vi "Test Array to Map.vi"() -> ()   [LabVIEW 2020]
uses:
  9a7eb577-90c4-4537-9fff-6973843e9f2b.vi
  9a7eb577-90c4-4537-9fff-6973843e9f2b.vi/b0178052-0c48-4c9a-874f-40b592e34ac5.vi
  <vilib>/addons/_JKI Toolkits/Caraya/classes/Assert/Assert Equal Value and Type_Variant.vi
  <vilib>/addons/_JKI Toolkits/Caraya/classes/Test/Test.lvclass
  <vilib>/addons/_JKI Toolkits/Caraya/classes/Assert/Assert.lvclass
panel:
  out "error out":errorcluster
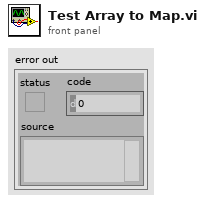
[diagram p1: front panel]
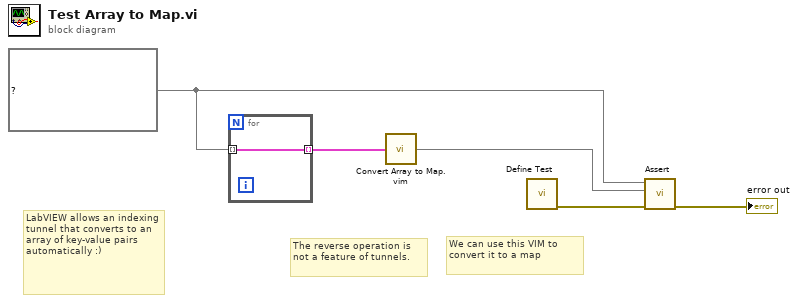
[diagram p0: block diagram]
diagram:
  w4 = map{i32, cluster{"bool":bool, "string":string}} {0={"bool"=FALSE, "string"="zero"}, 1={"bool"=TRUE, "string"="one"}} ("map out")
  # "We can use this VIM to convert it to a map"
  # "The reverse operation is not a feature of tunnels."
  # "LabVIEW allows an indexing tunnel that converts to an array of key-value pairs automatically :)"
  n1 = for {
    tunnel: [w6] -> w5 mode=indexing
    tunnel: w4 -> [w6] mode=indexing
  }
  n2 = call "Convert Array to Map.vim"("array"=w5) -> ("map"=w1:map{i32, cluster{"bool":bool, "string":string}})  [unwired: 6 in]
  n3 = call <vilib>:"Define Test.vi"() -> ("error out"=w2:errorcluster)  [unwired: 11 in]
  n4 = call-poly <vilib>:"Assert.vi"("error in (no error)"=w2, "Y"=w1, "X"=w4) -> ("error out"=→"error out":errorcluster)  [unwired: 8 in]
